vi "W32B Find Node Terminal.vi"(0 "VI reference":refnum<vi>, 5 "node class":string, 7 "source?":bool, 11 "error in":errorcluster) -> (4 "terminal":refnum<vi>, 15 "error out":errorcluster)   [LabVIEW 2020]
doc: "Finds the first node of class node class on the top-level block diagram of the VI behind VI reference and returns its first terminal whose direction matches source? - TRUE for an output terminal, FALSE for an input terminal."
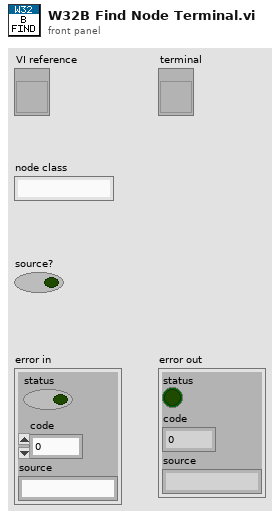
[diagram p1: front panel]
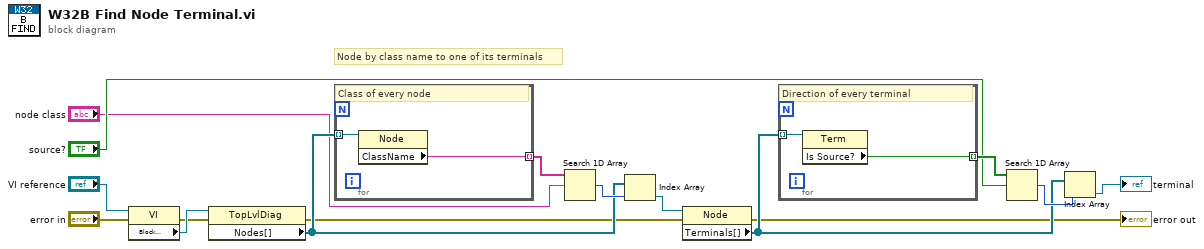
[diagram p0: block diagram]
diagram:
  # "Node by class name to one of its terminals"
  n1 = property class="VI"(reference="VI reference", error in="error in") -> (error out=w7:errorcluster, "Block Diagram"=w8:refnum<vi>)  [unwired: 1 out]
  n2 = property class="TopLvlDiag"(reference=w8, error in=w7) -> (error out=w9:errorcluster, "Nodes[]"=w10:refnum<vi>[])  [unwired: 1 out]
  n3 = for {
    tunnel: w10 -> [w17] mode=indexing
    tunnel: [w18] -> w11 mode=indexing
    # "Class of every node"
    n4 = property class="Node"(reference=w17) -> ("ClassName"=w18:string)  [unwired: 1 in, 2 out]
  }
  n5 = Search 1D Array(1D array=w11, element="node class") -> (index of element=w12:i32)  [unwired: 1 in]
  n6 = Index Array(array=w10, index=w12) -> (element=w13:refnum<vi>)
  n7 = property class="Node"(reference=w13, error in=w9) -> (error out=→"error out":errorcluster, "Terminals[]"=w14:refnum<vi>[])  [unwired: 1 out]
  n8 = for {
    tunnel: w14 -> [w19] mode=indexing
    tunnel: [w20] -> w15 mode=indexing
    # "Direction of every terminal"
    n9 = property class="Term"(reference=w19) -> ("Is Source?"=w20:bool)  [unwired: 1 in, 2 out]
  }
  n10 = Search 1D Array(1D array=w15, element="source?") -> (index of element=w16:i32)  [unwired: 1 in]
  n11 = Index Array(array=w14, index=w16) -> (element=→"terminal":refnum<vi>)
